vi "Initialize Error Map.vi"(8 "error in (no error)":errorcluster, 11 "Modbus in":refnum<class "Modbus.lvclass">) -> (0 "error out":errorcluster, 3 "Modbus out":refnum<class "Modbus.lvclass">)   [LabVIEW 2026, in "Modbus.lvlib" / "Modbus.lvclass"]
uses:
  Modbus.lvclass
  Modbus.lvclass/Modbus.ctl
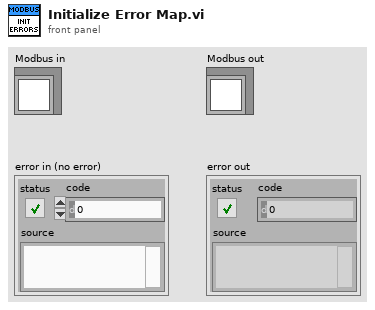
[diagram p1: front panel]
types:
  T1 = cluster{"Status":bool, "Code":i32, "Message":string}[]
  T2 = map{i32, cluster{"Status":bool, "Message":string}}
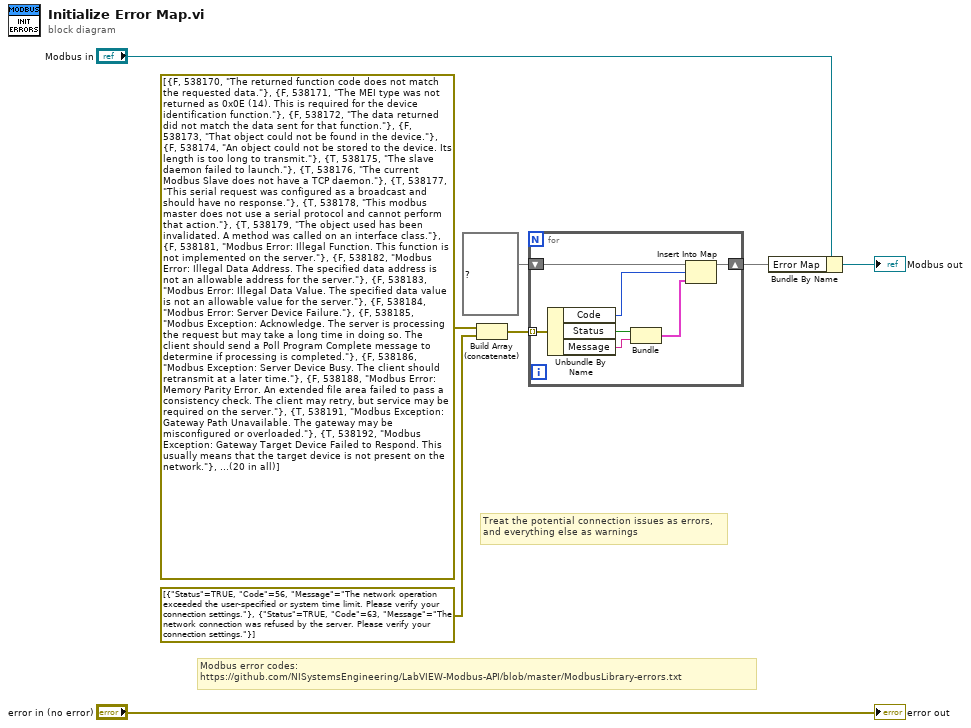
[diagram p0: block diagram]
diagram:
  # "Treat the potential connection issues as errors,\nand everything else as warnings"
  # "Modbus error codes:\nhttps://github.com/NISystemsEngineering/LabVIEW-Modbus-API/blob/master/ModbusLibrary-errors.txt"
  n1 = Build Array (concatenate)(T1 [{"Status"=FALSE, "Code"=538170, "Message"="The returned function code does not match the requested data."}, {"Status"=FALSE, "Code"=538171, "Message"="The MEI type was not returned as 0x0E (14). This is required for the device identification function."}, {"Status"=FALSE, "Code"=538172, "Message"="The data returned did not match the data sent for that function."}, {"Status"=FALSE, "Code"=538173, "Message"="That object could not be found in the device."}, {"Status"=FALSE, "Code"=538174, "Message"="An object could not be stored to the device. Its length is too long to transmit."}, {"Status"=TRUE, "Code"=538175, "Message"="The slave daemon failed to launch."}, {"Status"=TRUE, "Code"=538176, "Message"="The current Modbus Slave does not have a TCP daemon."}, {"Status"=TRUE, "Code"=538177, "Message"="This serial request was configured as a broadcast and should have no response."}, {"Status"=TRUE, "Code"=538178, "Message"="This modbus master does not use a serial protocol and cannot perform that action."}, {"Status"=TRUE, "Code"=538179, "Message"="The object used has been invalidated. A method was called on an interface class."}, {"Status"=FALSE, "Code"=538181, "Message"="Modbus Error: Illegal Function. This function is not implemented on the server."}, {"Status"=FALSE, "Code"=538182, "Message"="Modbus Error: Illegal Data Address. The specified data address is not an allowable address for the server."}, {"Status"=FALSE, "Code"=538183, "Message"="Modbus Error: Illegal Data Value. The specified data value is not an allowable value for the server."}, {"Status"=FALSE, "Code"=538184, "Message"="Modbus Error: Server Device Failure."}, {"Status"=FALSE, "Code"=538185, "Message"="Modbus Exception: Acknowledge. The server is processing the request but may take a long time in doing so. The client should send a Poll Program Complete message to determine if processing is completed."}, {"Status"=FALSE, "Code"=538186, "Message"="Modbus Exception: Server Device Busy. The client should retransmit at a later time."}, {"Status"=FALSE, "Code"=538188, "Message"="Modbus Error: Memory Parity Error. An extended file area failed to pass a consistency check. The client may retry, but service may be required on the server."}, {"Status"=TRUE, "Code"=538191, "Message"="Modbus Exception: Gateway Path Unavailable. The gateway may be misconfigured or overloaded."}, {"Status"=TRUE, "Code"=538192, "Message"="Modbus Exception: Gateway Target Device Failed to Respond. This usually means that the target device is not present on the network."}, {"Status"=TRUE, "Code"=538193, "Message"="Modbus Exception: Response Transaction ID doesn't match Request. This usually occurs on network error."}], T1 [{"Status"=TRUE, "Code"=56, "Message"="The network operation exceeded the user-specified or system time limit. Please verify your connection settings."}, {"Status"=TRUE, "Code"=63, "Message"="The network connection was refused by the server. Please verify your connection settings."}]) -> (w5:T1)
  n2 = for {
    tunnel: w5 -> [w15] mode=indexing
    shift-right: [w12] -> w3
    shift-left: T2 {} ("map out") -> [w13]
    n3 = Unbundle By Name(w15) -> ("Code"=w14:i32, "Status"=w11:bool, "Message"=w10:string)
    n4 = Bundle("Status"=w11, "Message"=w10) -> (w9:cluster{"Status":bool, "Message":string})  [unwired: 1 in]
    n5 = Insert Into Map(map in=w13, key=w14, value=w9) -> (map out=w12:T2)  [unwired: 2 out]
  }
  n6 = Bundle By Name(cluster="Modbus in", "Error Map"=w3) -> (→"Modbus out":refnum<class "Modbus.lvclass">)
  "error out" <- "error in (no error)"
